vi "Injecting Report Class.vi"() -> ()   [LabVIEW 2020]
uses:
  classes/Test Suite/Define Test Suite (JUnit Report).vi
  classes/Test Suite/Test Suite.lvclass
panel:
  in  "Report Path":path
  out "error out":errorcluster
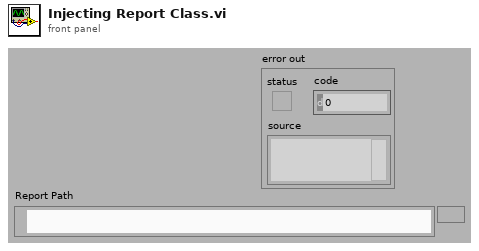
[diagram p1: front panel]
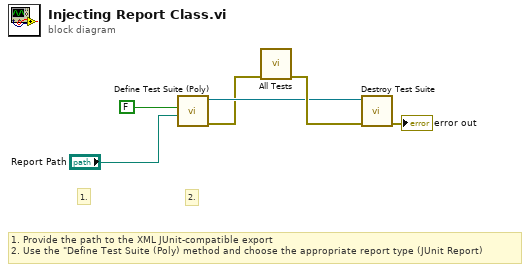
[diagram p0: block diagram]
diagram:
  # "2."
  # "1."
  # "1. Provide the path to the XML JUnit-compatible export\n2. Use the \"Define Test Suite (Poly) method and choose the appropriate report type (JUnit Report)"
  n1 = call-poly "Define Test Suite (Poly).vi"("Report Path"="Report Path", "Interactive"=FALSE) -> ("error out"=w3:errorcluster, "Test Suite"=w4:refnum<class "Test Suite.lvclass">)  [unwired: 7 in, 1 out]
  n2 = call "All Tests.vi"("error in (no error)"=w3) -> ("error out"=w6:errorcluster)  [unwired: 10 in]
  n3 = call-dynamic "Destroy Test Suite.vi"("error in (no error)"=w6, "Test Suite in"=w4) -> ("error out"=→"error out":errorcluster)  [unwired: 8 in, 1 out]
